vi "HandShaking.vi"(6 "Elapsed Time":u32, 8 "error in":errorcluster, 9 "Sequence Context":refnum<k7>, 10 "Stop":refnum<user-event>, 11 "TestExec":refnum<class "TestExec.lvclass">) -> (0 "error out":errorcluster, 3 "TestExec out":refnum<class "TestExec.lvclass">)   [LabVIEW 2025, in "TestExec.lvclass"]
uses:
  TestExec.lvclass
  C:/Working copy/TS Manager/Plugin/Tests/Submodule EOL/TS Execution Interface/OPC UA/Abstract.lvclass
  TestExec.lvclass/TestExec.ctl
  40e5e5ce-79b7-40ff-98c1-3a323906afd5.vi
  OPC UA/Read Rx from PLC.vi
  OPC UA/Read Tx to PLC.vi
  <vilib>/addons/TestStand/_TSUtility.llb/TestStand - Get Property Value (Number {Signed 32-bit Integer}).vi
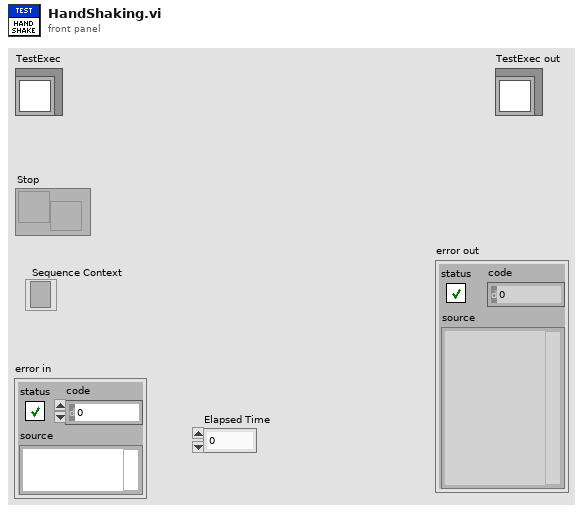
[diagram p1: front panel]
types:
  T1 = typedef "OPC UA.lvlib/OPC UA.lvclass/Tester Tx Dataset.ctl" = cluster{"Fault":bool, "StepNo":u32, "Ready":bool, "HighVoltage":bool, "TestRunning":bool, "ResultsReady":bool, "Results":u32, "ElapsedTime":u32, "Online":bool, "TimeCompleted":i32[], "Timeout":bool, "Heartbeat":bool}
  T2 = typedef "OPC UA.lvlib/OPC UA.lvclass/Tester Rx Dataset.ctl" = cluster{"Start":bool, "NestStatus":bool, "PalletID":u32, "BarcodeData":string, "StepEcho":u32, "Cylinder_1":bool, "Cylinder_2":bool, "Cylinder_3":bool, "Cylinder_4":bool, "Cylinder_5":bool, "ResultsAck":bool, "Reset":bool, "Stop":bool, "FaultCode":u32}
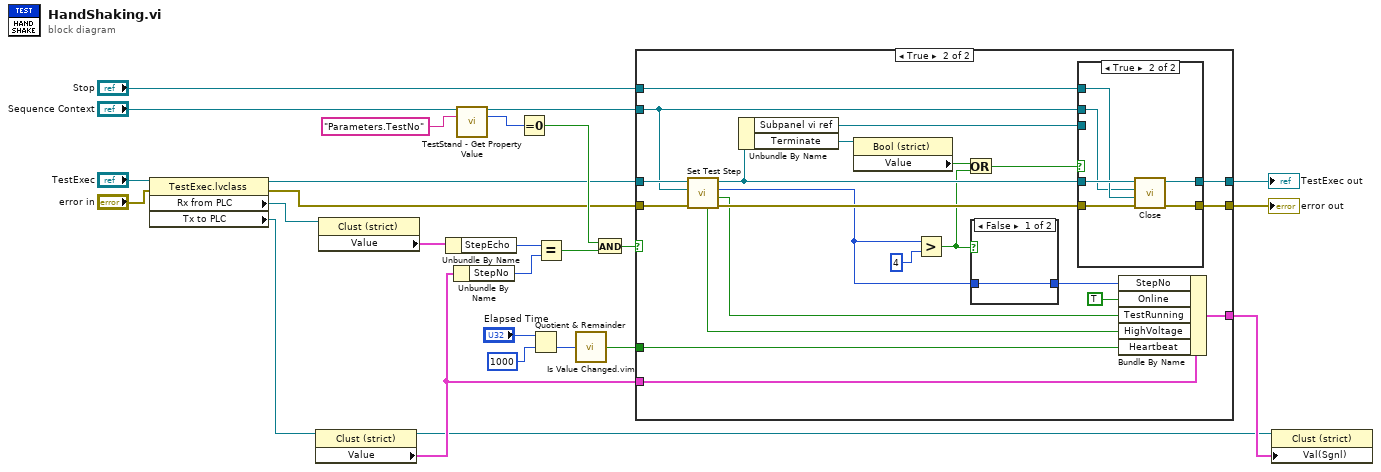
[diagram p0: block diagram]
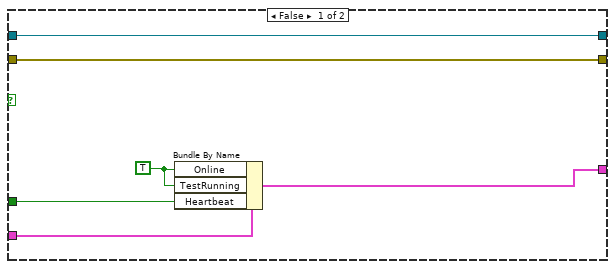
[diagram p2: hidden frame]
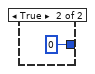
[diagram p3: hidden frame]
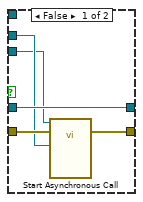
[diagram p4: hidden frame]
diagram:
  n1 = property class="TestExec.lvclass"(reference="TestExec", error in="error in") -> (reference out=w2:refnum<class "TestExec.lvclass">, error out=w3:errorcluster, "Rx from PLC"=w4:refnum<vi>, "Tx to PLC"=w5:refnum<vi>)
  n2 = property on="Property Node" class="Clust (strict)"(reference=w5) -> (reference out=w6:refnum<vi>, "Value"=w7:T1)  [unwired: 1 in, 1 out]
  n3 = property on="Property Node" class="Clust (strict)"(reference=w4) -> ("Value"=w26:T2)  [unwired: 1 in, 2 out]
  n4 = Unbundle By Name(w26) -> ("StepEcho"=w12:u32)
  n5 = Unbundle By Name(w7) -> ("StepNo"=w11:u32)
  n6 = call-poly <vilib>:"TestStand - Get Property Value.vi"("Sequence Context In"="Sequence Context", "Lookup String"="Parameters.TestNo") -> ("Sequence Context Out"=w1:refnum<k7>, "Value"=w23:i32)  [unwired: 11 in, 1 out]
  n7 = Equal To 0?(x=w23) -> (x = 0?=w9:bool)
  n8 = Quotient & Remainder(x="Elapsed Time", y=u32 1000) -> (floor(x/y)=w19:u32)  [unwired: 1 out]
  n9 = Equal?(x=w12, y=w11) -> (x = y?=w8:bool)
  n10 = call "Is Value Changed.vim"("value"=w19) -> ("changed or first call?"=w17:bool)
  n11 = And(x=w9, y=w8) -> (x .and. y?=w24:bool)
  n12 = case shown="True" w24 {
    tunnel: w7 -> [w31 w41]
    tunnel: w1 -> [_ w36]
    tunnel: "Stop" -> [_ w50]
    tunnel: w2 -> [w32 w53]
    tunnel: [w32 w51] -> w21
    tunnel: w17 -> [w28 w40]
    tunnel: [w30 w37] -> w16
    tunnel: [w27 w48] -> w15
    tunnel: w3 -> [w27 w47]
    frame False {
      w29 = TRUE ("Online")
      n13 = Bundle By Name(cluster=w31, "Online"=w29, "TestRunning"=w29, "Heartbeat"=w28) -> (w30:T1)
    }
    frame True {
      n14 = call "Set Test Step .vi"("error in"=w47, "Sequence Context In"=w36, "TestExec.lvclass"=w53) -> ("error out"=w49:errorcluster, "Test Running"=w39:bool, "Next Step"=w34:i32, "TestExec.lvclass"=w46:refnum<class "TestExec.lvclass">, "HV"=w38:bool)  [unwired: 4 in]
      n15 = Unbundle By Name(w46) -> ("Subpanel vi ref"=w45:refnum<vi>, "Terminate"=w44:refnum<vi>)
      n16 = property class="Bool (strict)"(reference=w44) -> ("Value"=w43:bool)  [unwired: 1 in, 2 out]
      n17 = Greater?(x=w34, y=4) -> (0:w35:bool)
      n18 = Or(x=w43, y=w35) -> (x .or. y?=w42:bool)
      n19 = case shown="False" w35 {
        tunnel: w34 -> [w55 _]
        tunnel: [w55 0 ("Next Step")] -> w33
        frame False {
        }
        frame True {
        }
      }
      n20 = case shown="True" w42 {
        tunnel: w46 -> [w61 w67]
        tunnel: [w61 w66] -> w51
        tunnel: w50 -> [_ w65]
        tunnel: w36 -> [w58 w64]
        tunnel: w49 -> [w60 w63]
        tunnel: [w59 w62] -> w48
        tunnel: w45 -> [w57 _]
        frame False {
          n21 = call-by-ref "Start Asynchronous Call"(reference=w57, error in=w60, "Sequence Context"=w58) -> (error out=w59:errorcluster)  [unwired: 10 in, 2 out]
        }
        frame True {
          n22 = call-dynamic "Close.vi"("error in"=w63, "Stop Event"=w65, "Sequence Context"=w64, "TestExec in"=w67) -> ("error out"=w62:errorcluster, "TestExec out"=w66:refnum<class "TestExec.lvclass">)  [unwired: 6 in]
        }
      }
      n23 = Bundle By Name(cluster=w41, "StepNo"=w33, "Online"=TRUE, "TestRunning"=w39, "HighVoltage"=w38, "Heartbeat"=w40) -> (w37:T1)
    }
  }
  "error out" <- w15
  "TestExec out" <- w21
  n24 = property on="Property Node" class="Clust (strict)"(reference=w6, "Val(Sgnl)"=w16) -> ()  [unwired: 1 in, 2 out]
